vi "GlobalMenuStatusStorage.vi"(1 "Read/Write":bool, 2 "Cluster":cluster{}, 3 "Device":string) -> ()   [LabVIEW 2024]
panel:
  out "Cluster 2":cluster{}
  # "usually ip"
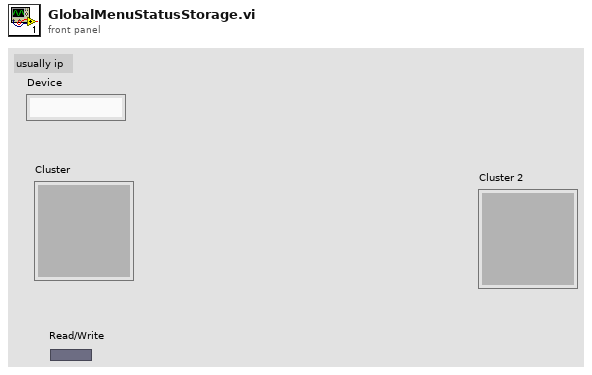
[diagram p1: front panel]
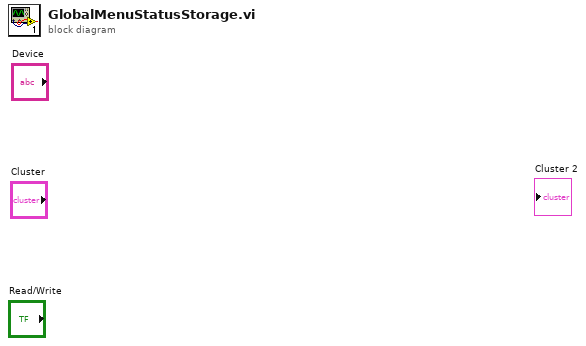
[diagram p0: block diagram]
diagram:
